vi "m3to reception.vi"   [LabVIEW 2017]
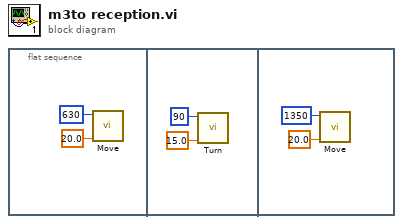
[diagram p0: block diagram]
diagram:
  n1 = flat-sequence {
    frame #0 {
      n2 = call "Move.vi"("Speed (0-30)"=20.0, "Distance (mm)"=630) -> ()  [unwired: 8 in]
    }
    frame #1 {
      n3 = call "Turn.vi"("Speed (0-30)"=15.0, "Angle (degrees)"=90) -> ()  [unwired: 10 in]
    }
    frame #2 {
      n4 = call "Move.vi"("Speed (0-30)"=20.0, "Distance (mm)"=1350) -> ()  [unwired: 8 in]
    }
  }
